vi "VIH ProjFile - Item Rule - Convert Paths.vi"(7 "Root Dir":path, 10 "Operation":enum16{"Read", "Write"}(ring), 11 "Item Rule":T1) -> (3 "Item Rule out":T1)   [LabVIEW 2014]
doc: "::: VI Helpeks :::\nCopyright (c) 2000-2026 Konstantin Shifershteyn. All rights reserved."
uses:
  _VIH HelpGen.llb/VIH HelpGen Typedef - Cluster - File Rule.ctl
  _VIH HelpGen.llb/VIH HelpGen Typedef - Enum - Default,Enable,Disable.ctl
  _VIH HelpGen.llb/VIH HelpGen Typedef - Cluster - File Rule - Source Paths.ctl
  _VIH HelpGen.llb/VIH HelpGen Typedef - Cluster - File Rule - Target Paths.ctl
  _VIH HelpGen.llb/VIH HelpGen Typedef - Enum - Description Mode.ctl
  _VIH HelpGen.llb/VIH HelpGen Typedef - Cluster - Control Rule.ctl
  _VIH HelpGen.llb/VIH HelpGen Typedef - Cluster - Enum Value Info.ctl
  _VIH HelpGen.llb/VIH HelpGen Typedef - Cluster - Group Rule - Flags.ctl
panel:
  # "VI Helpeks\nCopyright (c) 2012-2026 Konstantin Shifershteyn"
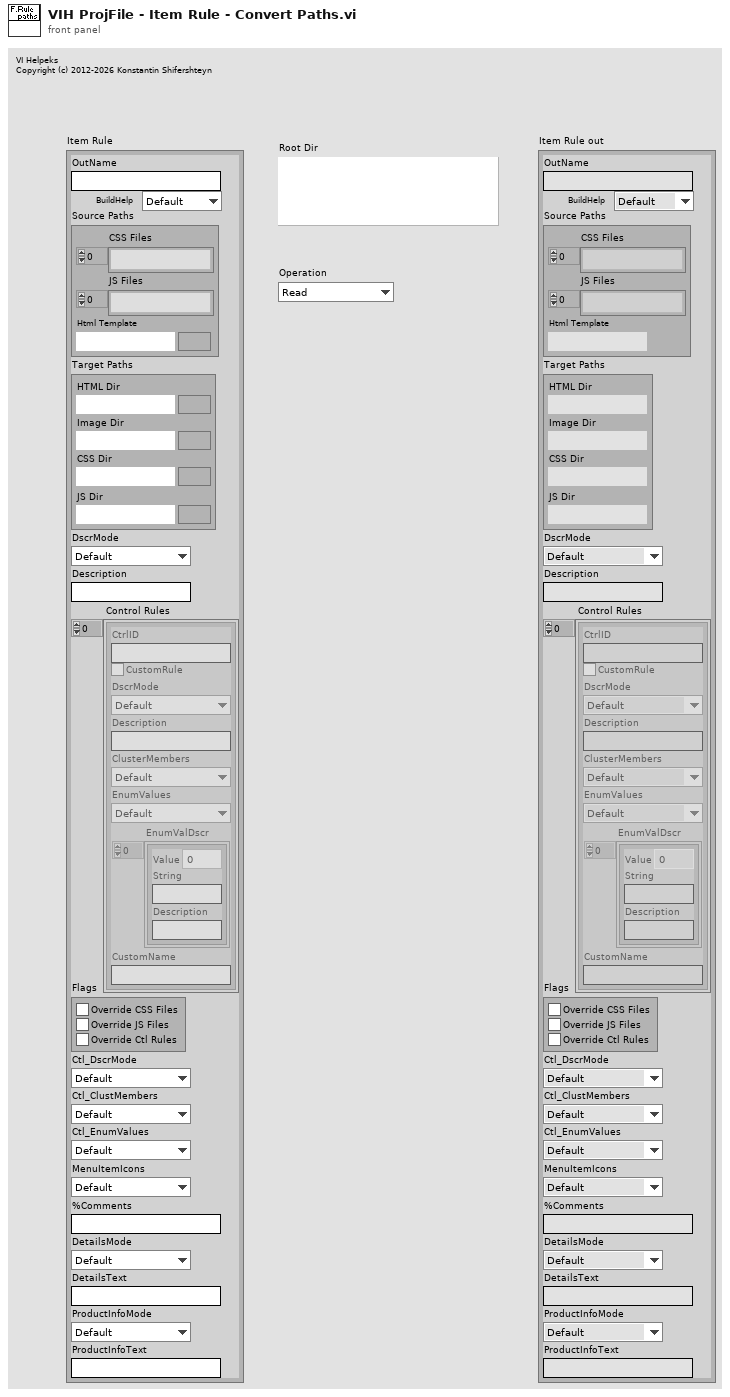
[diagram p1: front panel]
types:
  T1 = typedef "VIH HelpGen Typedef - Cluster - File Rule.ctl" = cluster{"OutName":string, "BuildHelp":T2, "Source Paths":T3, "Target Paths":T4, "DscrMode":T5, "Description":string, "Control Rules":T6[], "Flags":T8, "Ctl_DscrMode":T5, "Ctl_ClustMembers":T2, "Ctl_EnumValues":T2, "MenuItemIcons":T2, "%Comments":string, "DetailsMode":T5, "DetailsText":string, "ProductInfoMode":T2, "ProductInfoText":string}
  T2 = typedef "VIH HelpGen Typedef - Enum - Default,Enable,Disable.ctl" = enum16{"Default", "Enable", "Disable"}
  T3 = typedef "VIH HelpGen Typedef - Cluster - File Rule - Source Paths.ctl" = cluster{"CSS Files":path[], "JS Files":path[], "Html Template":path}
  T4 = typedef "VIH HelpGen Typedef - Cluster - File Rule - Target Paths.ctl" = cluster{"HTML Dir":path, "Image Dir":path, "CSS Dir":path, "JS Dir":path}
  T5 = typedef "VIH HelpGen Typedef - Enum - Description Mode.ctl" = enum16{"Default", "Description", "Description1", "Description2", "Custom", "None"}
  T6 = typedef "VIH HelpGen Typedef - Cluster - Control Rule.ctl" = cluster{"CtrlID":string, "CustomRule":bool, "DscrMode":T5, "Description":string, "ClusterMembers":T2, "EnumValues":T2, "EnumValDscr":T7[], "CustomName":string}
  T7 = typedef "VIH HelpGen Typedef - Cluster - Enum Value Info.ctl" = cluster{"Value":ext, "String":string, "Description":string}
  T8 = typedef "VIH HelpGen Typedef - Cluster - Group Rule - Flags.ctl" = cluster{"Override CSS Files":bool, "Override JS Files":bool, "Override Ctl Rules":bool}
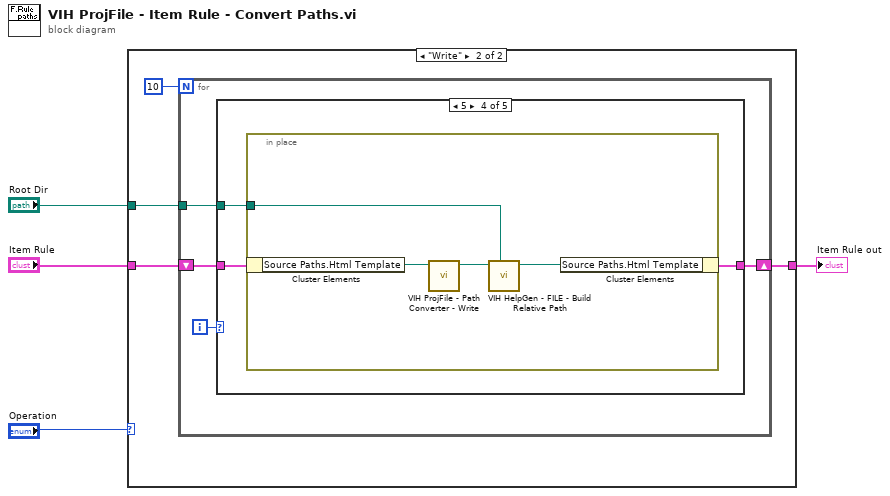
[diagram p0: block diagram]
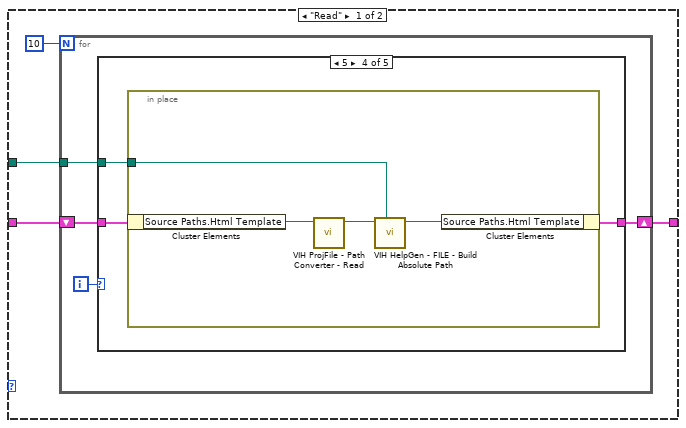
[diagram p2: hidden frame]
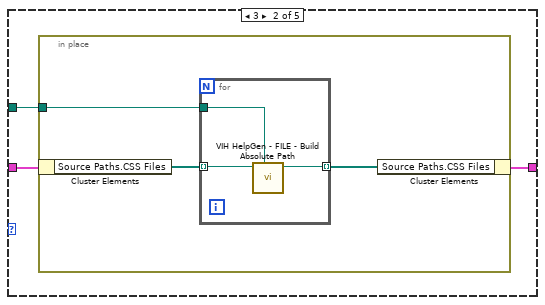
[diagram p4: hidden frame]
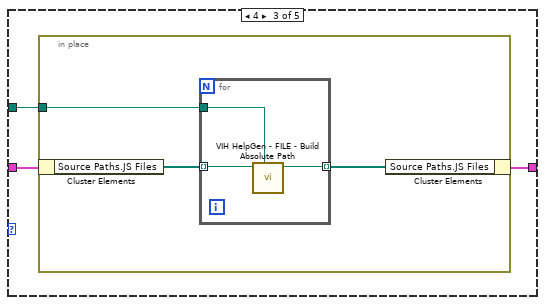
[diagram p5: hidden frame]
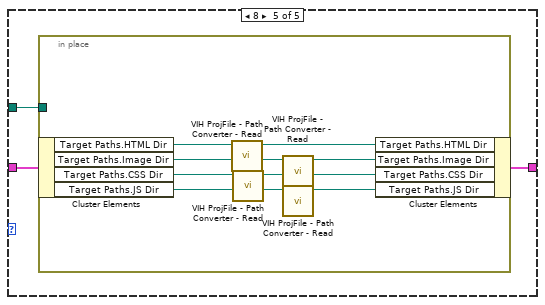
[diagram p6: hidden frame]
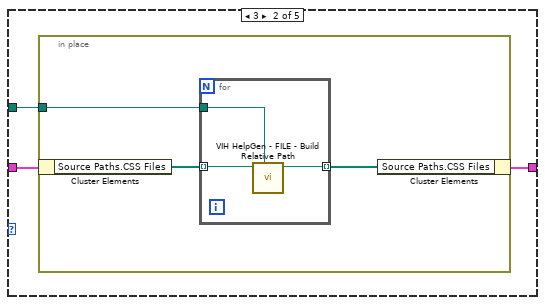
[diagram p8: hidden frame]
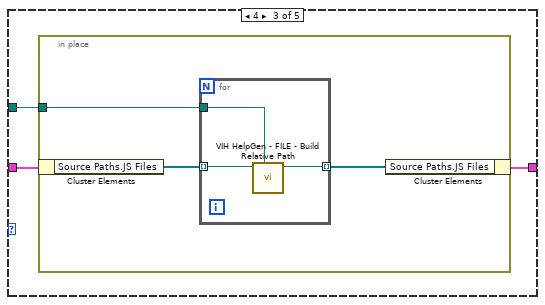
[diagram p9: hidden frame]
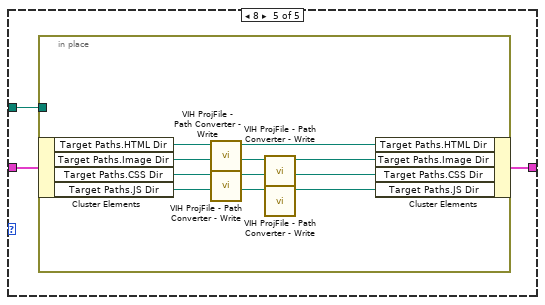
[diagram p10: hidden frame]
diagram:
  n1 = case shown="\"Write\"" "Operation" {
    tunnel: "Item Rule" -> [w8 w53]
    tunnel: [w7 w52] -> w3
    tunnel: "Root Dir" -> [w5 w50]
    frame "Read" {
      n2 = for {
        N: 10 -> [_]
        shift-right: [w11] -> w7
        shift-left: w8 -> [w10]
        tunnel: w5 -> [w9]
        i -> [w12]
        n3 = case shown="5" w12 {
          tunnel: [w13 w15 w24 w33 w40] -> w11
          tunnel: w10 -> [w13 w16 w25 w34 w41]
          tunnel: w9 -> [_ w14 w23 w32 w39]
          frame Default {
          }
          frame 3 {
            n4 = in-place {
              in-place-border: w14 -> [w18]
              n5 = in-place-cluster #1(w16) -> ("Source Paths.CSS Files"=w19:path[])
              n6 = for {
                tunnel: w19 -> [w22] mode=indexing
                tunnel: w18 -> [w21]
                tunnel: [w20] -> w17 mode=indexing
                n7 = call "VIH HelpGen - FILE - Build Absolute Path.vi"("Root Path"=w21, "Path in"=w22) -> ("Path out"=w20:path)  [unwired: 9 in]
              }
              n8 = in-place-cluster #1("Source Paths.CSS Files"=w17) -> (w15:T1)
            }
          }
          frame 4 {
            n9 = in-place {
              in-place-border: w23 -> [w27]
              n10 = in-place-cluster #2(w25) -> ("Source Paths.JS Files"=w28:path[])
              n11 = for {
                tunnel: w28 -> [w31] mode=indexing
                tunnel: w27 -> [w30]
                tunnel: [w29] -> w26 mode=indexing
                n12 = call "VIH HelpGen - FILE - Build Absolute Path.vi"("Root Path"=w30, "Path in"=w31) -> ("Path out"=w29:path)  [unwired: 9 in]
              }
              n13 = in-place-cluster #2("Source Paths.JS Files"=w26) -> (w24:T1)
            }
          }
          frame 5 {
            n14 = in-place {
              in-place-border: w32 -> [w38]
              n15 = in-place-cluster #3(w34) -> ("Source Paths.Html Template"=w36:path)
              n16 = call "VIH ProjFile - Path Converter - Read.vi"("Path in"=w36) -> ("Path out"=w35:path)  [unwired: 10 in]
              n17 = call "VIH HelpGen - FILE - Build Absolute Path.vi"("Root Path"=w38, "Path in"=w35) -> ("Path out"=w37:path)  [unwired: 9 in]
              n18 = in-place-cluster #3("Source Paths.Html Template"=w37) -> (w33:T1)
            }
          }
          frame 8 {
            n19 = in-place {
              in-place-border: w39 -> [_]
              n20 = in-place-cluster #4(w41) -> ("Target Paths.HTML Dir"=w49:path, "Target Paths.Image Dir"=w47:path, "Target Paths.CSS Dir"=w45:path, "Target Paths.JS Dir"=w43:path)
              n21 = call "VIH ProjFile - Path Converter - Read.vi"("Path in"=w49) -> ("Path out"=w48:path)  [unwired: 10 in]
              n22 = call "VIH ProjFile - Path Converter - Read.vi"("Path in"=w45) -> ("Path out"=w44:path)  [unwired: 10 in]
              n23 = call "VIH ProjFile - Path Converter - Read.vi"("Path in"=w47) -> ("Path out"=w46:path)  [unwired: 10 in]
              n24 = call "VIH ProjFile - Path Converter - Read.vi"("Path in"=w43) -> ("Path out"=w42:path)  [unwired: 10 in]
              n25 = in-place-cluster #4("Target Paths.HTML Dir"=w48, "Target Paths.Image Dir"=w46, "Target Paths.CSS Dir"=w44, "Target Paths.JS Dir"=w42) -> (w40:T1)
            }
          }
        }
      }
    }
    frame "Write" {
      n26 = for {
        N: 10 -> [_]
        shift-right: [w56] -> w52
        shift-left: w53 -> [w55]
        tunnel: w50 -> [w54]
        i -> [w57]
        n27 = case shown="5" w57 {
          tunnel: [w58 w60 w69 w78 w85] -> w56
          tunnel: w55 -> [w58 w61 w70 w79 w86]
          tunnel: w54 -> [_ w59 w68 w77 w84]
          frame Default {
          }
          frame 3 {
            n28 = in-place {
              in-place-border: w59 -> [w63]
              n29 = in-place-cluster #5(w61) -> ("Source Paths.CSS Files"=w64:path[])
              n30 = for {
                tunnel: w64 -> [w67] mode=indexing
                tunnel: w63 -> [w66]
                tunnel: [w65] -> w62 mode=indexing
                n31 = call "VIH HelpGen - FILE - Build Relative Path.vi"("Root Path"=w66, "Path in"=w67) -> ("Path out"=w65:path)  [unwired: 9 in]
              }
              n32 = in-place-cluster #5("Source Paths.CSS Files"=w62) -> (w60:T1)
            }
          }
          frame 4 {
            n33 = in-place {
              in-place-border: w68 -> [w72]
              n34 = in-place-cluster #6(w70) -> ("Source Paths.JS Files"=w73:path[])
              n35 = for {
                tunnel: w73 -> [w76] mode=indexing
                tunnel: w72 -> [w75]
                tunnel: [w74] -> w71 mode=indexing
                n36 = call "VIH HelpGen - FILE - Build Relative Path.vi"("Root Path"=w75, "Path in"=w76) -> ("Path out"=w74:path)  [unwired: 9 in]
              }
              n37 = in-place-cluster #6("Source Paths.JS Files"=w71) -> (w69:T1)
            }
          }
          frame 5 {
            n38 = in-place {
              in-place-border: w77 -> [w83]
              n39 = in-place-cluster #7(w79) -> ("Source Paths.Html Template"=w81:path)
              n40 = call "VIH ProjFile - Path Converter - Write.vi"("Path in"=w81) -> ("Path out"=w80:path)  [unwired: 10 in]
              n41 = call "VIH HelpGen - FILE - Build Relative Path.vi"("Root Path"=w83, "Path in"=w80) -> ("Path out"=w82:path)  [unwired: 9 in]
              n42 = in-place-cluster #7("Source Paths.Html Template"=w82) -> (w78:T1)
            }
          }
          frame 8 {
            n43 = in-place {
              in-place-border: w84 -> [_]
              n44 = in-place-cluster #8(w86) -> ("Target Paths.HTML Dir"=w94:path, "Target Paths.Image Dir"=w92:path, "Target Paths.CSS Dir"=w90:path, "Target Paths.JS Dir"=w88:path)
              n45 = call "VIH ProjFile - Path Converter - Write.vi"("Path in"=w94) -> ("Path out"=w93:path)  [unwired: 10 in]
              n46 = call "VIH ProjFile - Path Converter - Write.vi"("Path in"=w90) -> ("Path out"=w89:path)  [unwired: 10 in]
              n47 = call "VIH ProjFile - Path Converter - Write.vi"("Path in"=w92) -> ("Path out"=w91:path)  [unwired: 10 in]
              n48 = call "VIH ProjFile - Path Converter - Write.vi"("Path in"=w88) -> ("Path out"=w87:path)  [unwired: 10 in]
              n49 = in-place-cluster #8("Target Paths.HTML Dir"=w93, "Target Paths.Image Dir"=w91, "Target Paths.CSS Dir"=w89, "Target Paths.JS Dir"=w87) -> (w85:T1)
            }
          }
        }
      }
    }
  }
  "Item Rule out" <- w3
